vi "RT Init.vi"(6 "Device Outputs FIFO":refnum<k33>, 8 "error in":errorcluster, 11 "Device Ref":T13=18446744073709551615 format="%.0x") -> (0 "error out":errorcluster, 3 "RT Data":T1={"Timekeeper hdl"="", "clkDisc session"=variant, "Compiled Data"={"SyncMod?"=FALSE, "SyncMod"="", "ConnectionSettings"={"Mode"=enum."Generate sample clock", "pxitrig"=FALSE, "pfi0"=FALSE, "pfi1"=FALSE, "pfi2"=FALSE, "External Pin"=enum."PFI0", "Routes"=[]}, "TimeKeeper"="", "ScanOffset(%)"=0.0, "StartDelay(s)"=0, "Time Ref Settings"={"Time Reference"=enum."GPS", "Priority 1"=0, "Priority 2"=0, "IRIG type"=enum."IRIGB AM", "Terminal"="", "PPSSetTime"=FALSE, "Start Time"=timestamp(0 s since 1904-01-01)}, "FIFO Locations"={"BoardTime"=[], "Status"=[]}}, "OutputsData"=[], "OutputsFIFO"=refnum, "Scan Period"=0, "Timekeeper type"=enum."6683", "SyncMod type"=enum."6683", "SyncMod hdl"="", "Custom Device Name"=""} {"Compiled Data"."Time Ref Settings"."Priority 2" min=0 max=255; "Compiled Data"."Time Ref Settings"."Priority 1" min=0 max=255}, 4 "Name":string)   [LabVIEW 2020, in "NI Synchronization Engine.lvlib"]
uses:
  NI Synchronization Engine.lvlib
  <vilib>/NI VeriStand/Custom Device API/Custom Device Item Ref.ctl
  RT Data Cluster.ctl
  mdevClkDisc.llb/_clkDisc_session.ctl
  Shared/Compiled Data.ctl
  Shared/Connection Settings.ctl
  Shared/Mode.ctl
  Shared/External Pin.ctl
  Shared/Routes.ctl
  Shared/Route.ctl
  Shared/Time Ref Settings.ctl
  Shared/Time Reference.ctl
  Shared/IRIG Type.ctl
  timekeeper type.ctl
  Shared/Constants.vi
  <vilib>/NI VeriStand/Custom Device API/Get Item Property (Variant).vi
  <instrlib>/niSync/niSync.llb/niSync Initialize (Default).vi
  <vilib>/NI VeriStand/Custom Device API/Custom Device API.lvlib
  Shared/NI Synchronization Shared.lvlib
  <vilib>/NI VeriStand/Custom Device Tools/Custom Device Utility Library/Custom Device Utility Library.lvlib
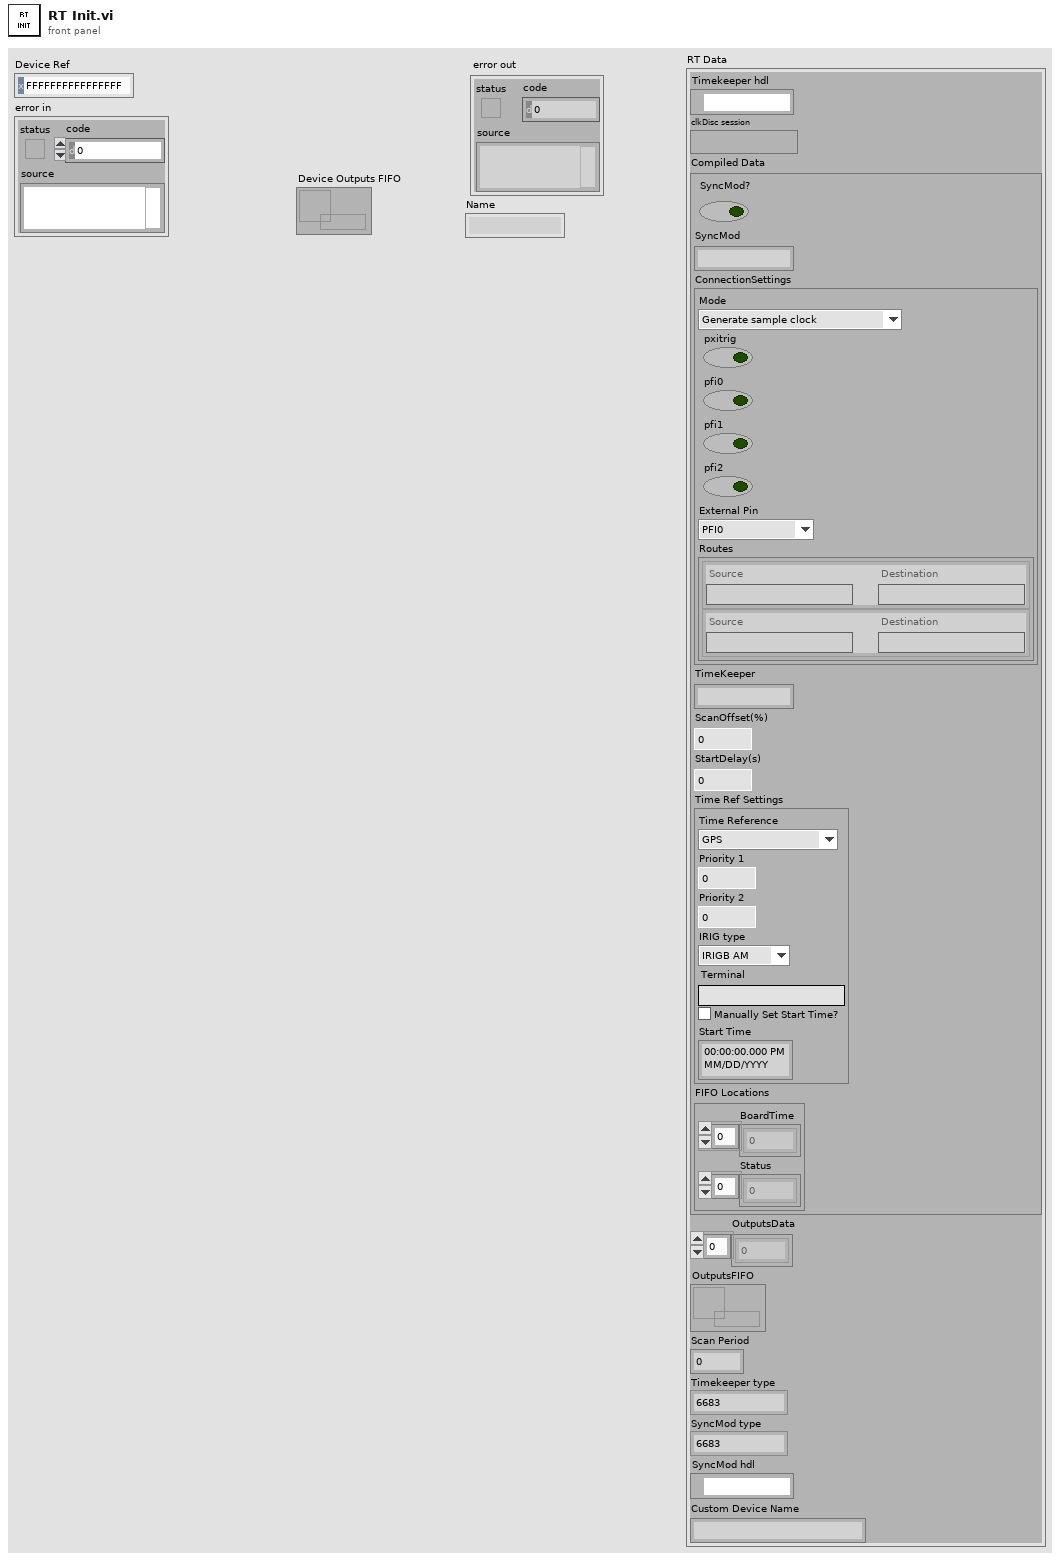
[diagram p1: front panel]
types:
  T1 = typedef "NI Synchronization Engine.lvlib/RT Data Cluster.ctl" = cluster{"Timekeeper hdl":refnum<k15>, "clkDisc session":T2, "Compiled Data":T3, "OutputsData":dbl[], "OutputsFIFO":refnum<k33>, "Scan Period":u32, "Timekeeper type":T12, "SyncMod type":T12, "SyncMod hdl":refnum<k15>, "Custom Device Name":string}
  T2 = typedef "_clkDisc_session.ctl" = variant
  T3 = typedef "NI Synchronization Shared.lvlib/Compiled Data.ctl" = cluster{"SyncMod?":bool, "SyncMod":string, "ConnectionSettings":T4, "TimeKeeper":string, "ScanOffset(%)":dbl, "StartDelay(s)":u16, "Time Ref Settings":T9, "FIFO Locations":cluster{"BoardTime":i32[], "Status":i32[]}}
  T4 = typedef "NI Synchronization Shared.lvlib/Connection Settings.ctl" = cluster{"Mode":T5, "pxitrig":bool, "pfi0":bool, "pfi1":bool, "pfi2":bool, "External Pin":T6, "Routes":T7}
  T5 = typedef "NI Synchronization Shared.lvlib/Mode.ctl" = enum16{"Generate sample clock", "Route sample clock out of chassis", "Route sample clock into chassis", "Custom routes"}
  T6 = typedef "NI Synchronization Shared.lvlib/External Pin.ctl" = enum16{"PFI0", "PFI1", "PFI2"}
  T7 = typedef "NI Synchronization Shared.lvlib/Routes.ctl" = T8[]
  T8 = typedef "NI Synchronization Shared.lvlib/Route.ctl" = cluster{"Source":string, "Destination":string}
  T9 = typedef "NI Synchronization Shared.lvlib/Time Ref Settings.ctl" = cluster{"Time Reference":T10, "Priority 1":i32, "Priority 2":i32, "IRIG type":T11, "Terminal":string, "PPSSetTime":bool, "Start Time":timestamp}
  T10 = typedef "NI Synchronization Shared.lvlib/Time Reference.ctl" = enum16{"GPS", "IRIG", "PPS", "1588 Ordinary Clock", "802.1AS", "PXI Chassis Clock", "Free Running (Internal)"}
  T11 = typedef "NI Synchronization Shared.lvlib/IRIG Type.ctl" = enum16{"IRIGB DC", "IRIGB AM"}
  T12 = typedef "NI Synchronization Engine.lvlib/timekeeper type.ctl" = enum16{"6683", "6683H", "6682", "6682H", "non-timekeeper", "timekeeper"}
  T13 = typedef "Custom Device API.lvlib/Custom Device Item Ref.ctl" = u64
  T14 = typedef "Custom Device API.lvlib/Custom Device Item Info.ctl" = cluster{"Name":string, "Is Channel":bool, "GUID":string, "Is Waveform":bool}
  T15 = typedef "Custom Device API.lvlib/Custom Device Channel.ctl" = cluster{"Type":T16, "Units":string, "Default Value":dbl, "Faultable":bool, "Scalable":bool}
  T16 = typedef "Custom Device API.lvlib/Custom Device Channel Type.ctl" = enum16{"Input", "Output"}
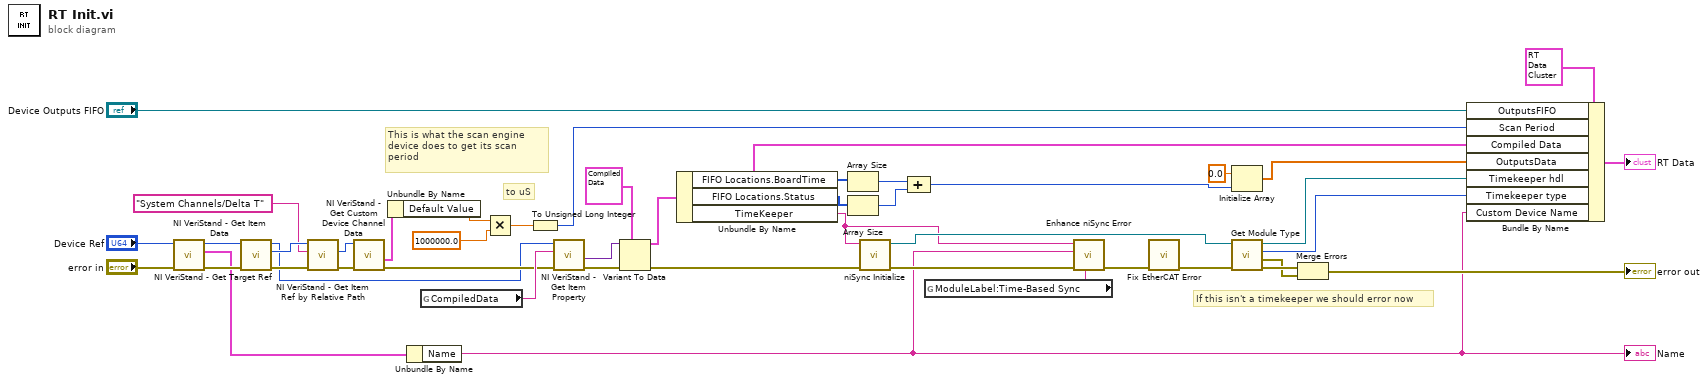
[diagram p0: block diagram]
diagram:
  # "If this isn't a timekeeper we should error now"
  # "This is what the scan engine device does to get its scan period"
  # "to uS"
  n1 = call <vilib>:"NI VeriStand - Get Item Data.vi"("error in (no error)"="error in", "Item Ref in"="Device Ref") -> ("error out"=w16:errorcluster, "Item Info"=w13:T14, "Item Ref out"=w14:T13)  [unwired: 6 in, 1 out]
  n2 = call <vilib>:"NI VeriStand - Get Target Ref.vi"("error in"=w16, "Item Ref in"=w14) -> ("error out"=w24:errorcluster, "Target Ref"=w25:T13, "Item Ref out"=w17:T13)  [unwired: 6 in, 1 out]
  n3 = call <vilib>:"NI VeriStand - Get Item Ref by Relative Path.vi"("error in"=w24, "Relative Item Path"="System Channels/Delta T", "Section Ref in"=w25) -> ("error out"=w21:errorcluster, "Item Ref"=w22:T13)  [unwired: 5 in, 2 out]
  n4 = call <vilib>:"NI VeriStand - Get Custom Device Channel Data.vi"("error in (no error)"=w21, "Channel Ref in"=w22) -> ("error out"=w18:errorcluster, "Channel"=w20:T15)  [unwired: 4 in, 4 out]
  n5 = Unbundle By Name(w20) -> ("Default Value"=w29:dbl)
  n6 = Unbundle By Name(w13) -> ("Name"=w1:string)
  "Name" <- w1
  n7 = global read "Constants.vi" "CompiledData"() -> (w45:string)
  n8 = Multiply(x=w29, y=1000000.0) -> (x*y=w27:dbl)
  n9 = To Unsigned Long Integer(number=w27) -> (unsigned 32bit integer=w19:u32)
  n10 = call-poly <vilib>:"NI VeriStand - Get Item Property.vi"("error in (no error)"=w18, "Property Name"=w45, "Item Ref in"=w17) -> ("error out"=w44:errorcluster, "Value"=w40:variant)  [unwired: 5 in, 2 out]
  n11 = Variant To Data(error in=w44, type=T3 {"SyncMod?"=FALSE, "SyncMod"="", "ConnectionSettings"={"Mode"=enum."Generate sample clock", "pxitrig"=FALSE, "pfi0"=FALSE, "pfi1"=FALSE, "pfi2"=FALSE, "External Pin"=enum."PFI0", "Routes"=[]}, "TimeKeeper"="", "ScanOffset(%)"=0.0, "StartDelay(s)"=0, "Time Ref Settings"={"Time Reference"=enum."GPS", "Priority 1"=0, "Priority 2"=0, "IRIG type"=enum."IRIGB AM", "Terminal"="", "PPSSetTime"=FALSE, "Start Time"=timestamp(0 s since 1904-01-01)}, "FIFO Locations"={"BoardTime"=[], "Status"=[]}} ("Compiled Data"), Variant=w40) -> (data=w38:T3, error out=w41:errorcluster)
  n12 = Unbundle By Name(w38) -> ("FIFO Locations.BoardTime"=w36:i32[], "FIFO Locations.Status"=w35:i32[], "TimeKeeper"=w3:string)
  n13 = Array Size(array=w36) -> (size(s)=w34:i32)
  n14 = Array Size(array=w35) -> (size(s)=w33:i32)
  n15 = call-poly <instrlib>:"niSync Initialize.vi"("error in (no error)"=w41, "resource name"=w3) -> ("error out"=w6:errorcluster, "instrument handle out"=w5:refnum<k15>)  [unwired: 8 in]
  n16 = Compound Arithmetic op=ADD(w34, w33) -> (w32:i32)
  n17 = global read "Constants.vi" "ModuleLabel:Time-Based Sync"() -> (w2:string)
  n18 = call "Enhance niSync Error.vi"("sync config label"=w2, "error in (no error)"=w6, "custom device name"=w1, "resource name"=w3) -> ("error out"=w4:errorcluster)  [unwired: 7 in]
  n19 = call "Fix EtherCAT Error.vi"("error in (no error)"=w4) -> ("error out"=w7:errorcluster)  [unwired: 10 in]
  n20 = Initialize Array(0.0 ("element"), w32) -> (w30:dbl[])
  n21 = call "Get Module Type.vi"("error in (no error)"=w7, "IVI Refnum in"=w5) -> ("error out"=w10:errorcluster, "timekeeper check error out"=w9:errorcluster, "Module type"=w11:T12, "IVI Refnum out"=w12:refnum<k15>)  [unwired: 6 in]
  n22 = Merge Errors(w10, w9) -> (→"error out":errorcluster)
  n23 = Bundle By Name(cluster=T1 {"Timekeeper hdl"="", "clkDisc session"=variant, "Compiled Data"={"SyncMod?"=FALSE, "SyncMod"="", "ConnectionSettings"={"Mode"=enum."Generate sample clock", "pxitrig"=FALSE, "pfi0"=FALSE, "pfi1"=FALSE, "pfi2"=FALSE, "External Pin"=enum."PFI0", "Routes"=[]}, "TimeKeeper"="", "ScanOffset(%)"=0.0, "StartDelay(s)"=0, "Time Ref Settings"={"Time Reference"=enum."GPS", "Priority 1"=0, "Priority 2"=0, "IRIG type"=enum."IRIGB AM", "Terminal"="", "PPSSetTime"=FALSE, "Start Time"=timestamp(0 s since 1904-01-01)}, "FIFO Locations"={"BoardTime"=[], "Status"=[]}}, "OutputsData"=[], "OutputsFIFO"=refnum, "Scan Period"=0, "Timekeeper type"=enum."6683", "SyncMod type"=enum."6683", "SyncMod hdl"="", "Custom Device Name"=""}, "OutputsFIFO"="Device Outputs FIFO", "Scan Period"=w19, "Compiled Data"=w38, "OutputsData"=w30, "Timekeeper hdl"=w12, "Timekeeper type"=w11, "Custom Device Name"=w1) -> (→"RT Data":T1)
